vi "Labview_trieur_balles.vi"(10 "Numeric":i32) -> ()   [LabVIEW 2017]
uses:
  enum_trieur_balle.ctl
  <vilib>/Platform/TimedLoop/XDataNode/XDataNode.xnode
  <vilib>/Platform/TimedLoop/XDataNode/nitl_modes.ctl
  <vilib>/Platform/TimedLoop/XDataNode/XDNodeRunTimeDep.lvlib
  <vilib>/Platform/TimedLoop/XDataNode/wakeup.ctl
  <vilib>/Platform/TimedLoop/XDataNode/timing_clust.ctl
panel:
  in  "delay rotation 6":i32=38000
  in  "delay rotation 5":i32=37000
  in  "delay rotation 4":i32=36000
  in  "delay rotation 3":i32=36500
  in  "delay rotation 2":i32=36000
  in  "delay rotation":i32=39000
  in  "x 2":i32=10000000
  in  "x":i32=10000000
  out "x+1 4":i32
  out "Couleur 4":bool
  out "Cluster 4":T1
  out "x+1 3":i32
  out "Couleur 3":bool
  out "Cluster 3":T1
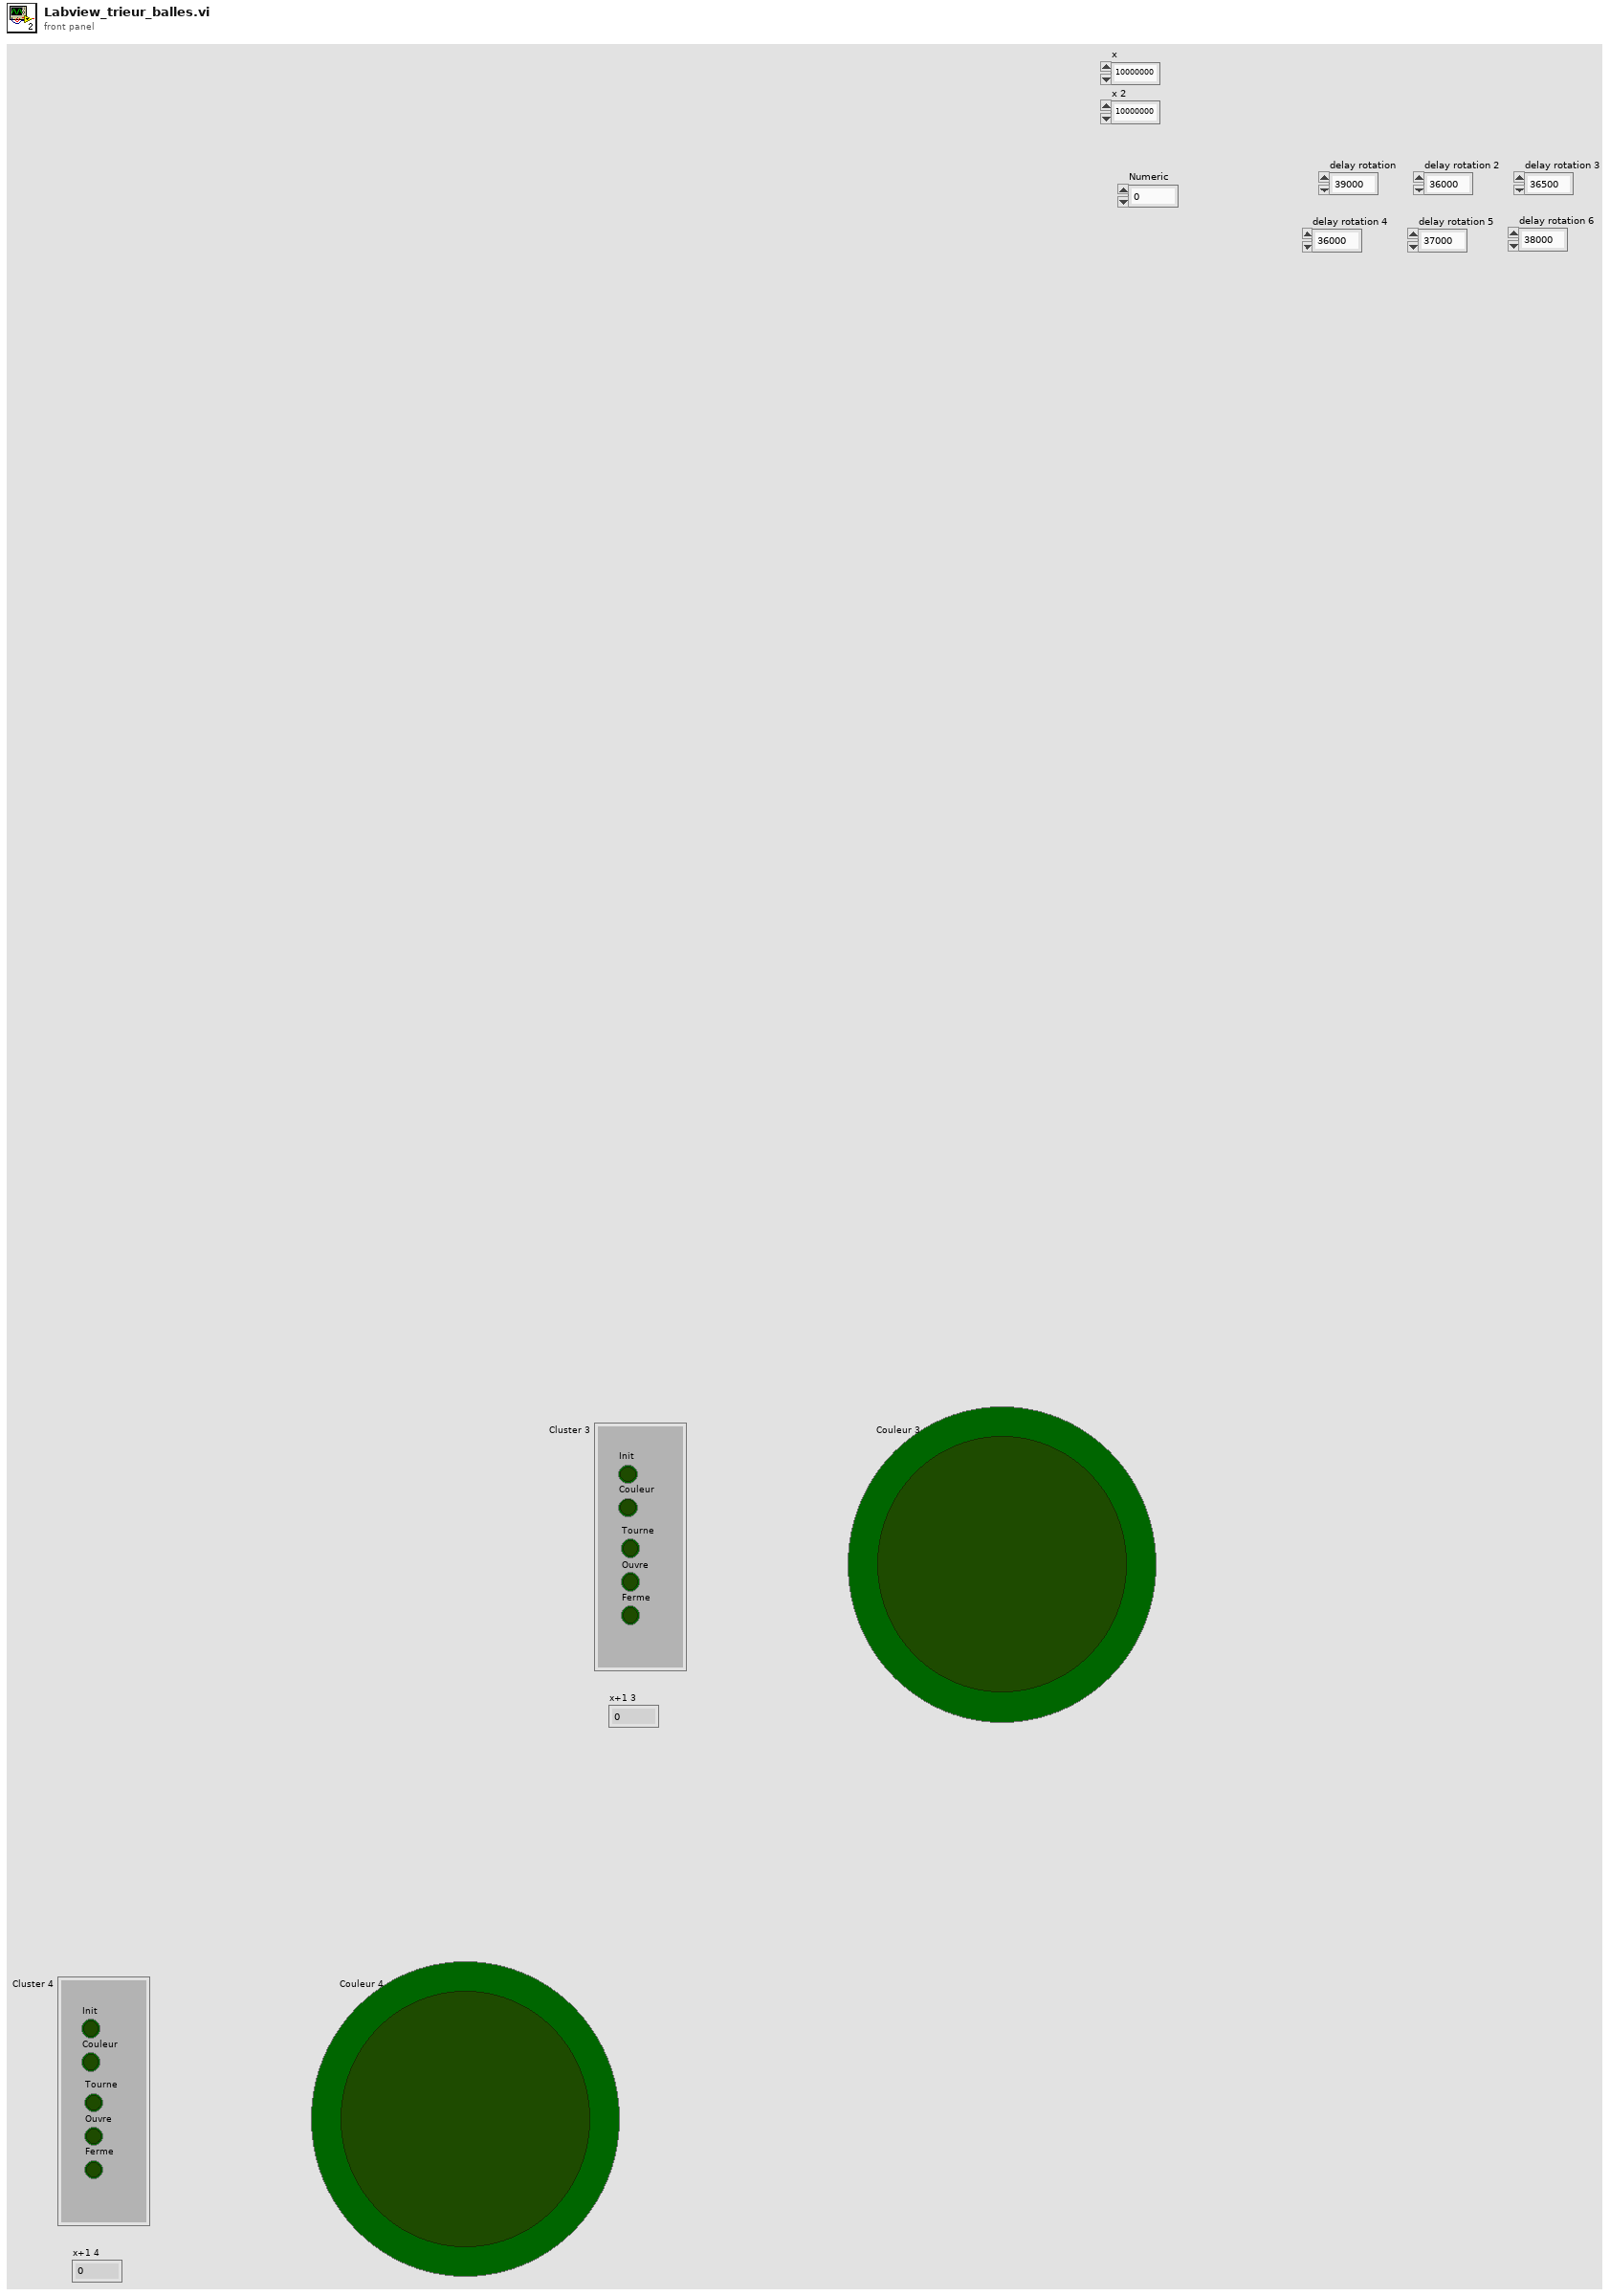
[diagram p1: front panel]
types:
  T1 = cluster{"Init":bool, "Couleur":bool, "Tourne":bool, "Ouvre":bool, "Ferme":bool}
  T2 = typedef "enum_trieur_balle.ctl" = enum16{"Initialisation", "Couleur", "Rotation", "Ouverture", "Fermeture"}
  T3 = cluster{"Booléen":bool, "Booléen 2":bool, "Booléen 3":bool, "Booléen 4":bool, "Booléen 5":bool}
  T4 = typedef "XDNodeRunTimeDep.lvlib/timing_clust.ctl" = cluster{"Expected End [f-1]":u64, "Actual End [f-1]":u64, "Finished Late? [f-1]":bool, "Expected End [i-1]":u64, "Actual End [i-1]":u64, "Finished Late? [i-1]":bool, "Expected Start [i]":u64, "Actual Start [i]":u64, "Expected Start [f]":u64, "Actual Start [f]":u64, "Source Name":string, "Structure Name":string, "Period":i64, "Deadline":i64, "Offset":i64, "Start":i64, "Priority":i32, "Timeout":i32, "Mode":T5, "Wakeup Reason":T6, "Error":errorcluster, "Source Type":string, "Secondary Source Type":string, "Global End Time":u64, "Global Start Time":u64, "Frame Duration":u64, "Iteration Duration":u64, "Assigned CPU":i32, "I/O Scan Engine Mode":u32}
  T5 = typedef "XDNodeRunTimeDep.lvlib/nitl_modes.ctl" = enum32{"No Change", "Process missed periods, maintain original phase", "Discard missed periods, maintain original phase", "Process missed periods, ignore original phase", "Discard missed periods, ignore original phase"}
  T6 = typedef "XDNodeRunTimeDep.lvlib/wakeup.ctl" = enum32{"Normal", "Aborted", "Asynchronous wakeup", "Timing source error", "Timed loop error", "Timeout"}
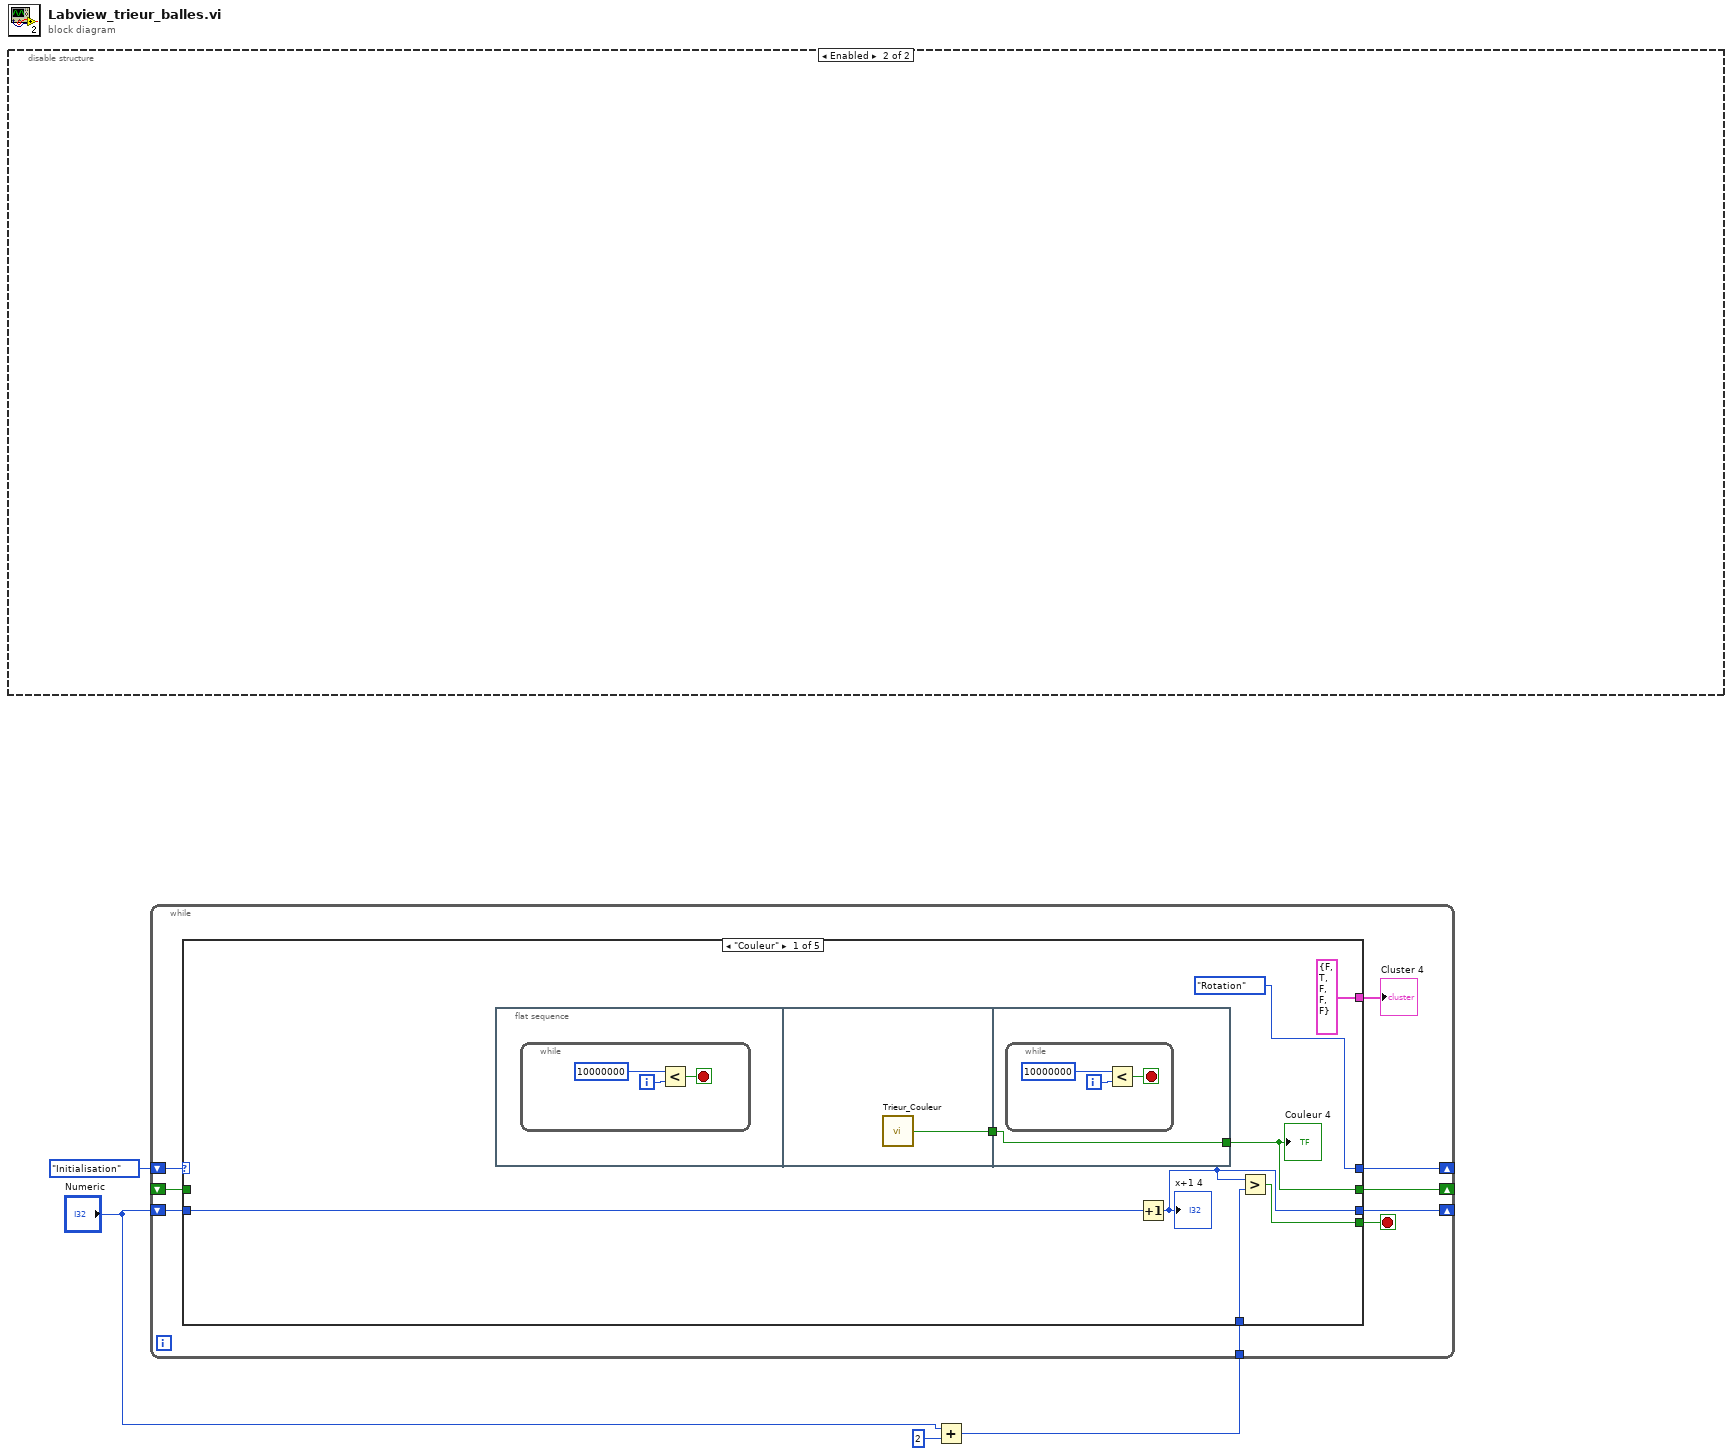
[diagram p0: block diagram]
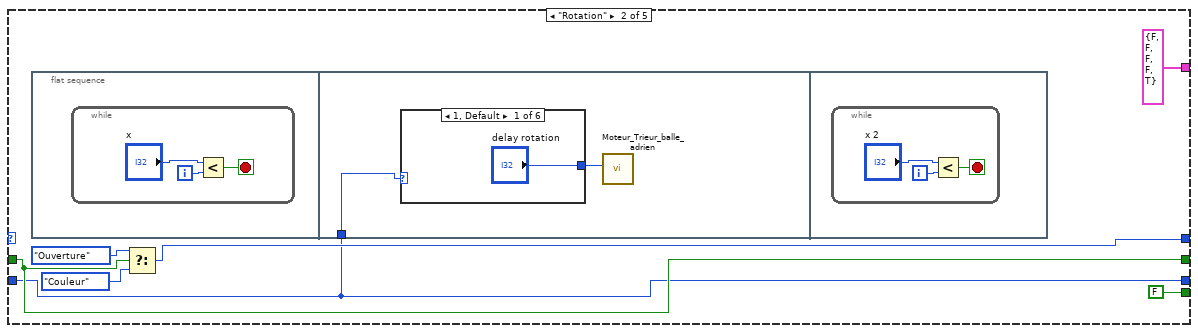
[diagram p2: hidden frame]
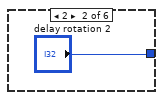
[diagram p3: hidden frame]
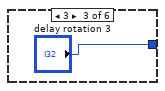
[diagram p4: hidden frame]
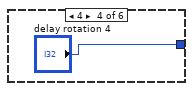
[diagram p5: hidden frame]
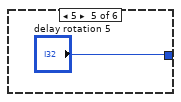
[diagram p6: hidden frame]
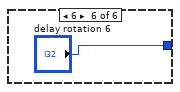
[diagram p7: hidden frame]
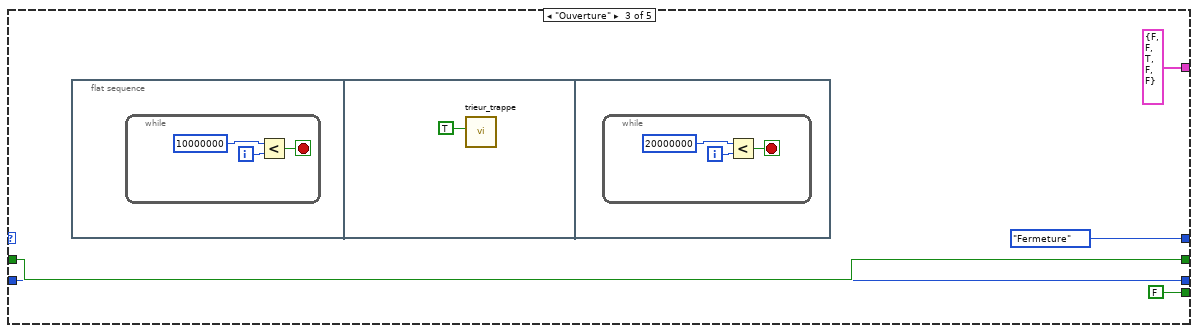
[diagram p8: hidden frame]
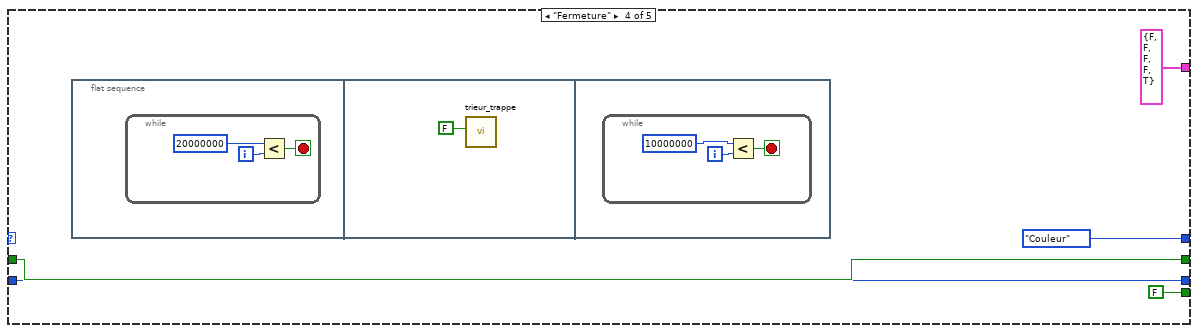
[diagram p9: hidden frame]
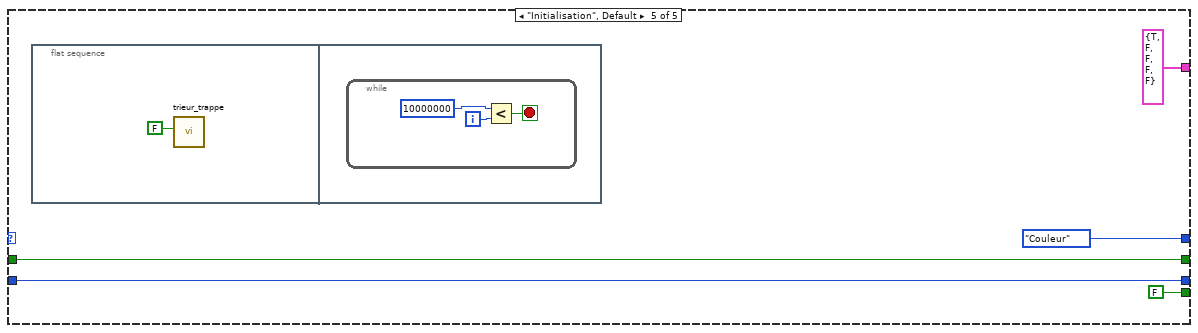
[diagram p10: hidden frame]
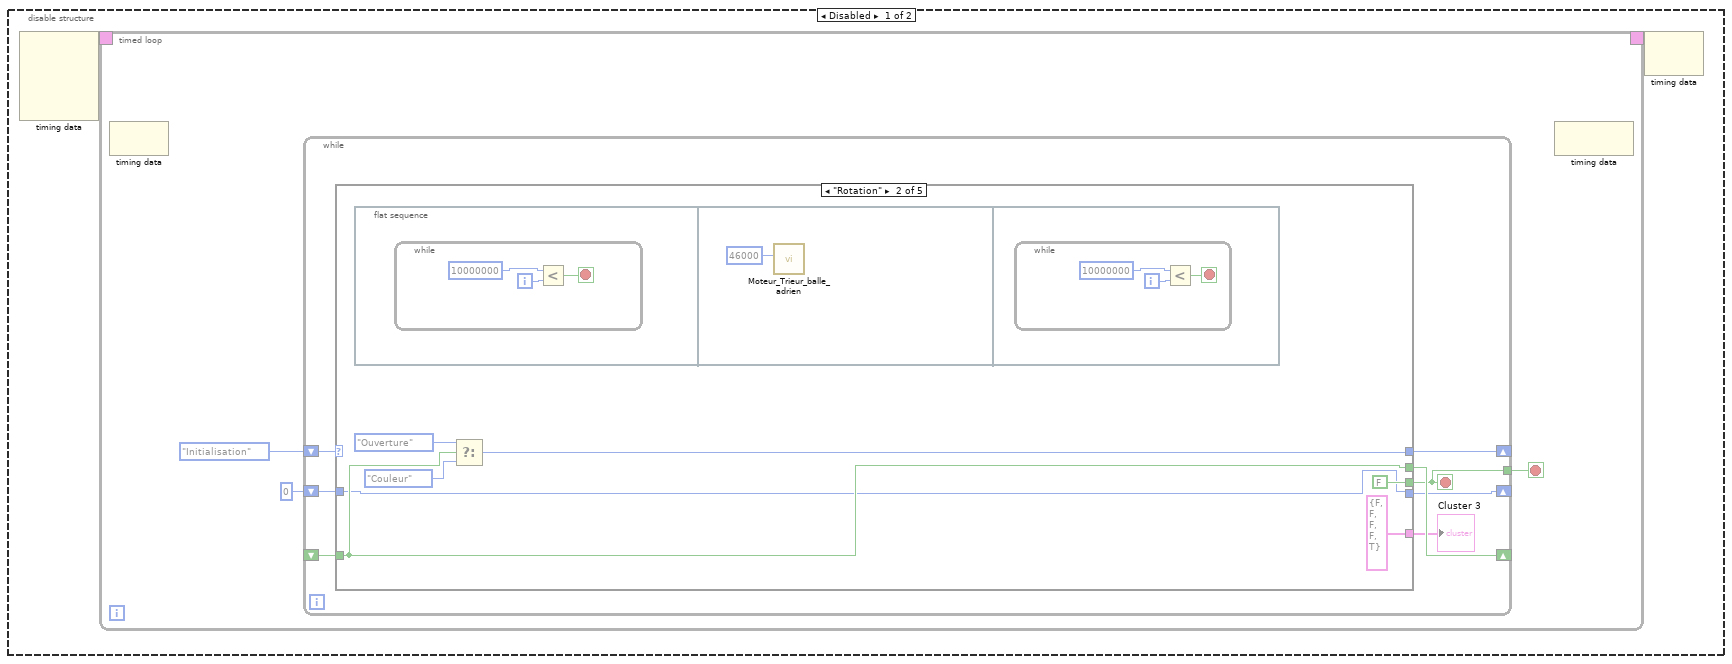
[diagram p11: hidden frame]
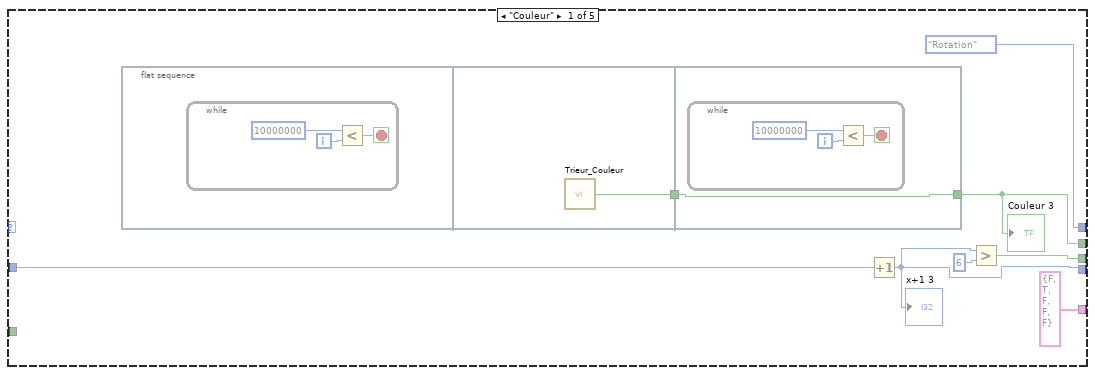
[diagram p12: hidden frame]
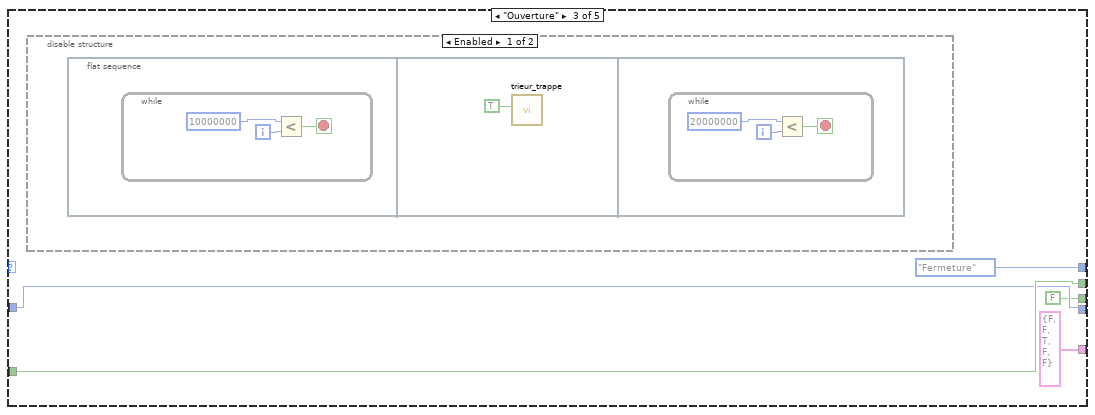
[diagram p13: hidden frame]
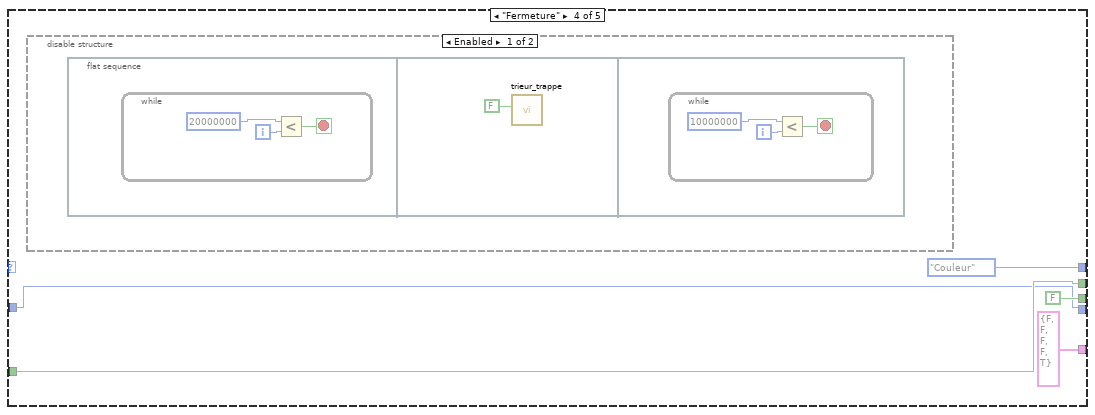
[diagram p15: hidden frame]
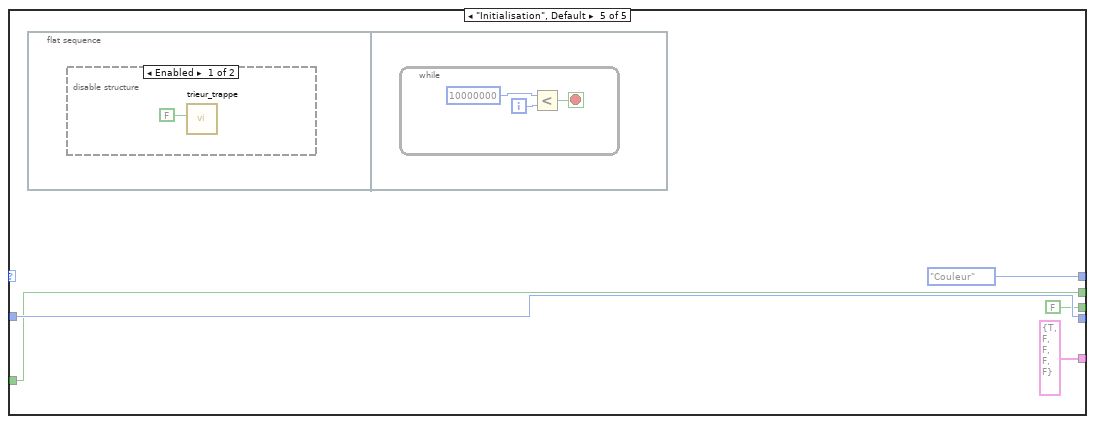
[diagram p17: hidden frame]
diagram:
  n1 = disable-structure shown="Enabled" {
    frame Disabled {
      n2 = node-c288() -> (w6:T4)  [unwired: 4 in]
      n3 = timed-loop {
        timing: w6 -> [_]
        timing-out: [_] -> w5
        stop <- w7 stop-if-true
        n4 = node-c288() -> ()  [unwired: 1 in, 1 out]
        n5 = while {
          shift-right: [w13] -> _
          shift-left: enum_trieur_balle."Initialisation" -> [w17]
          shift-right: [w16] -> _
          shift-left: _ -> [w12]
          shift-right: [w14] -> _
          shift-left: 0 -> [w15]
          tunnel: [w10] -> w7
          stop <- w10 stop-if-true
          n6 = case shown="\"Rotation\"" w17 {
            tunnel: [w19 w38 w52 w63 w73] -> w16
            tunnel: w15 -> [w25 w37 w51 w62 w76]
            tunnel: [w22 w37 w51 w62 w76] -> w14
            tunnel: [w20 FALSE FALSE FALSE FALSE] -> w10
            tunnel: [enum_trieur_balle."Rotation" w39 enum_trieur_balle."Fermeture" enum_trieur_balle."Couleur" enum_trieur_balle."Couleur"] -> w13
            tunnel: w12 -> [_ w38 w52 w63 w73]
            tunnel: [T3 {"Booléen"=FALSE, "Booléen 2"=TRUE, "Booléen 3"=FALSE, "Booléen 4"=FALSE, "Booléen 5"=FALSE} ("Cluster") T3 {"Booléen"=FALSE, "Booléen 2"=FALSE, "Booléen 3"=FALSE, "Booléen 4"=FALSE, "Booléen 5"=TRUE} ("Cluster") T3 {"Booléen"=FALSE, "Booléen 2"=FALSE, "Booléen 3"=TRUE, "Booléen 4"=FALSE, "Booléen 5"=FALSE} ("Cluster") T3 {"Booléen"=FALSE, "Booléen 2"=FALSE, "Booléen 3"=FALSE, "Booléen 4"=FALSE, "Booléen 5"=TRUE} ("Cluster") T3 {"Booléen"=TRUE, "Booléen 2"=FALSE, "Booléen 3"=FALSE, "Booléen 4"=FALSE, "Booléen 5"=FALSE} ("Cluster")] -> w11
            frame "Couleur" {
              n7 = flat-sequence {
                tunnel: [w29] -> w18
                tunnel: [w30] -> w19
                tunnel: w18 -> [w30]
                frame #0 {
                  n8 = while {
                    i -> [w28]
                    stop <- w26 stop-if-true
                    n9 = Less?(x=10000000, y=w28) -> (x < y?=w26:bool)
                  }
                }
                frame #1 {
                  n10 = call "Trieur_Couleur.vi"() -> ("Couleur"=w29:bool)  [unwired: 2 in]
                }
                frame #2 {
                  n11 = while {
                    i -> [w33]
                    stop <- w31 stop-if-true
                    n12 = Less?(x=10000000, y=w33) -> (x < y?=w31:bool)
                  }
                }
              }
              n13 = Increment(x=w25) -> (x+1=w22:i32)
              "x+1 3" <- w22
              n14 = Greater?(x=w22, y=6) -> (0:w20:bool)
              "Couleur 3" <- w19
            }
            frame "Rotation" {
              n15 = flat-sequence {
                frame #0 {
                  n16 = while {
                    i -> [w43]
                    stop <- w41 stop-if-true
                    n17 = Less?(x=10000000, y=w43) -> (x < y?=w41:bool)
                  }
                }
                frame #1 {
                  n18 = call "Moteur_Trieur_balle_adrien.vi"("delay rotation"=46000) -> ()  [unwired: 11 in]
                }
                frame #2 {
                  n19 = while {
                    i -> [w47]
                    stop <- w45 stop-if-true
                    n20 = Less?(x=10000000, y=w47) -> (x < y?=w45:bool)
                  }
                }
              }
              n21 = Select(t=enum_trieur_balle."Ouverture", s=w38, f=enum_trieur_balle."Couleur") -> (s? t:f=w39:T2)
            }
            frame "Ouverture" {
              n22 = disable-structure shown="Enabled" {
                frame Enabled {
                  n23 = flat-sequence {
                    frame #0 {
                      n24 = while {
                        i -> [w55]
                        stop <- w53 stop-if-true
                        n25 = Less?(x=10000000, y=w55) -> (x < y?=w53:bool)
                      }
                    }
                    frame #1 {
                      n26 = call "trieur_trappe.vi"("Ouvrir"=TRUE) -> ()  [unwired: 11 in]
                    }
                    frame #2 {
                      n27 = while {
                        i -> [w59]
                        stop <- w57 stop-if-true
                        n28 = Less?(x=20000000, y=w59) -> (x < y?=w57:bool)
                      }
                    }
                  }
                }
                frame Disabled {
                }
              }
            }
            frame "Fermeture" {
              n29 = disable-structure shown="Enabled" {
                frame Enabled {
                  n30 = flat-sequence {
                    frame #0 {
                      n31 = while {
                        i -> [w67]
                        stop <- w65 stop-if-true
                        n32 = Less?(x=20000000, y=w67) -> (x < y?=w65:bool)
                      }
                    }
                    frame #1 {
                      n33 = call "trieur_trappe.vi"("Ouvrir"=FALSE) -> ()  [unwired: 11 in]
                    }
                    frame #2 {
                      n34 = while {
                        i -> [w71]
                        stop <- w69 stop-if-true
                        n35 = Less?(x=10000000, y=w71) -> (x < y?=w69:bool)
                      }
                    }
                  }
                }
                frame Disabled {
                }
              }
            }
            frame "Initialisation", Default {
              n36 = flat-sequence {
                frame #0 {
                  n37 = disable-structure shown="Enabled" {
                    frame Enabled {
                      n38 = call "trieur_trappe.vi"("Ouvrir"=FALSE) -> ()  [unwired: 11 in]
                    }
                    frame Disabled {
                    }
                  }
                }
                frame #1 {
                  n39 = while {
                    i -> [w80]
                    stop <- w78 stop-if-true
                    n40 = Less?(x=10000000, y=w80) -> (x < y?=w78:bool)
                  }
                }
              }
            }
          }
          "Cluster 3" <- w11
        }
        n41 = node-c288() -> ()  [unwired: 1 in, 1 out]
      }
      n42 = node-c288(w5) -> ()  [unwired: 1 out]
    }
    frame Enabled {
    }
  }
  n43 = Add(x="Numeric", y=2) -> (x+y=w1:i32)
  n44 = while {
    shift-right: [w89] -> _
    shift-left: enum_trieur_balle."Initialisation" -> [w93]
    shift-right: [w92] -> _
    shift-left: _ -> [w88]
    shift-right: [w90] -> _
    shift-left: "Numeric" -> [w91]
    tunnel: w1 -> [w85]
    stop <- w86 stop-if-true
    n45 = case shown="\"Couleur\"" w93 {
      tunnel: [w96 w114 w135 w146 w156] -> w92
      tunnel: w91 -> [w101 w110 w134 w145 w159]
      tunnel: [w98 w110 w134 w145 w159] -> w90
      tunnel: [w97 FALSE FALSE FALSE FALSE] -> w86
      tunnel: [enum_trieur_balle."Rotation" w115 enum_trieur_balle."Fermeture" enum_trieur_balle."Couleur" enum_trieur_balle."Couleur"] -> w89
      tunnel: w88 -> [_ w114 w135 w146 w156]
      tunnel: [T3 {"Booléen"=FALSE, "Booléen 2"=TRUE, "Booléen 3"=FALSE, "Booléen 4"=FALSE, "Booléen 5"=FALSE} ("Cluster") T3 {"Booléen"=FALSE, "Booléen 2"=FALSE, "Booléen 3"=FALSE, "Booléen 4"=FALSE, "Booléen 5"=TRUE} ("Cluster") T3 {"Booléen"=FALSE, "Booléen 2"=FALSE, "Booléen 3"=TRUE, "Booléen 4"=FALSE, "Booléen 5"=FALSE} ("Cluster") T3 {"Booléen"=FALSE, "Booléen 2"=FALSE, "Booléen 3"=FALSE, "Booléen 4"=FALSE, "Booléen 5"=TRUE} ("Cluster") T3 {"Booléen"=TRUE, "Booléen 2"=FALSE, "Booléen 3"=FALSE, "Booléen 4"=FALSE, "Booléen 5"=FALSE} ("Cluster")] -> w87
      tunnel: w85 -> [w94 _ _ _ _]
      frame "Couleur" {
        n46 = flat-sequence {
          tunnel: [w105] -> w95
          tunnel: [w106] -> w96
          tunnel: w95 -> [w106]
          frame #0 {
            n47 = while {
              i -> [w104]
              stop <- w102 stop-if-true
              n48 = Less?(x=10000000, y=w104) -> (x < y?=w102:bool)
            }
          }
          frame #1 {
            n49 = call "Trieur_Couleur.vi"() -> ("Couleur"=w105:bool)  [unwired: 2 in]
          }
          frame #2 {
            n50 = while {
              i -> [w109]
              stop <- w107 stop-if-true
              n51 = Less?(x=10000000, y=w109) -> (x < y?=w107:bool)
            }
          }
        }
        n52 = Increment(x=w101) -> (x+1=w98:i32)
        "x+1 4" <- w98
        n53 = Greater?(x=w98, y=w94) -> (0:w97:bool)
        "Couleur 4" <- w96
      }
      frame "Rotation" {
        n54 = flat-sequence {
          tunnel: w110 -> [w120]
          frame #0 {
            n55 = while {
              i -> [w119]
              stop <- w118 stop-if-true
              n56 = Less?(x="x", y=w119) -> (x < y?=w118:bool)
            }
          }
          frame #1 {
            n57 = case shown="1, Default" w120 {
              tunnel: ["delay rotation" "delay rotation 2" "delay rotation 3" "delay rotation 4" "delay rotation 5" "delay rotation 6"] -> w121
              frame 1, Default {
              }
              frame 2 {
              }
              frame 3 {
              }
              frame 4 {
              }
              frame 5 {
              }
              frame 6 {
              }
            }
            n58 = call "Moteur_Trieur_balle_adrien.vi"("delay rotation"=w121) -> ()  [unwired: 11 in]
          }
          frame #2 {
            n59 = while {
              i -> [w130]
              stop <- w129 stop-if-true
              n60 = Less?(x="x 2", y=w130) -> (x < y?=w129:bool)
            }
          }
        }
        n61 = Select(t=enum_trieur_balle."Ouverture", s=w114, f=enum_trieur_balle."Couleur") -> (s? t:f=w115:T2)
      }
      frame "Ouverture" {
        n62 = flat-sequence {
          frame #0 {
            n63 = while {
              i -> [w138]
              stop <- w136 stop-if-true
              n64 = Less?(x=10000000, y=w138) -> (x < y?=w136:bool)
            }
          }
          frame #1 {
            n65 = call "trieur_trappe.vi"("Ouvrir"=TRUE) -> ()  [unwired: 11 in]
          }
          frame #2 {
            n66 = while {
              i -> [w142]
              stop <- w140 stop-if-true
              n67 = Less?(x=20000000, y=w142) -> (x < y?=w140:bool)
            }
          }
        }
      }
      frame "Fermeture" {
        n68 = flat-sequence {
          frame #0 {
            n69 = while {
              i -> [w150]
              stop <- w148 stop-if-true
              n70 = Less?(x=20000000, y=w150) -> (x < y?=w148:bool)
            }
          }
          frame #1 {
            n71 = call "trieur_trappe.vi"("Ouvrir"=FALSE) -> ()  [unwired: 11 in]
          }
          frame #2 {
            n72 = while {
              i -> [w154]
              stop <- w152 stop-if-true
              n73 = Less?(x=10000000, y=w154) -> (x < y?=w152:bool)
            }
          }
        }
      }
      frame "Initialisation", Default {
        n74 = flat-sequence {
          frame #0 {
            n75 = call "trieur_trappe.vi"("Ouvrir"=FALSE) -> ()  [unwired: 11 in]
          }
          frame #1 {
            n76 = while {
              i -> [w163]
              stop <- w161 stop-if-true
              n77 = Less?(x=10000000, y=w163) -> (x < y?=w161:bool)
            }
          }
        }
      }
    }
    "Cluster 4" <- w87
  }
